vi "Timer_New.vi"(8 "Pass_Through_Time":dbl=-1.0 format="%33.4f") -> (3 "TIMER":T1 {"Accumulated TIme" format="%13.5p"; "StartTime" format="%13.5p"})   [LabVIEW 2019, in "Trajectory_Library.lvlib"]
doc: "Creates and initializes a Timer data cluster.\n\nOutputs:\n - Timer -- The initialized Timer data cluster"
uses:
  Trajectory_Library.lvlib
  TypeDef/TIMER.ctl
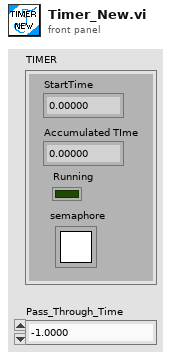
[diagram p1: front panel]
types:
  T1 = typedef "Trajectory_Library.lvlib/TIMER.ctl" = cluster{"StartTime":dbl, "Accumulated TIme":dbl, "Running":bool, "semaphore":T2}
  T2 = typedef "Semaphore RefNum" = refnum<k1>
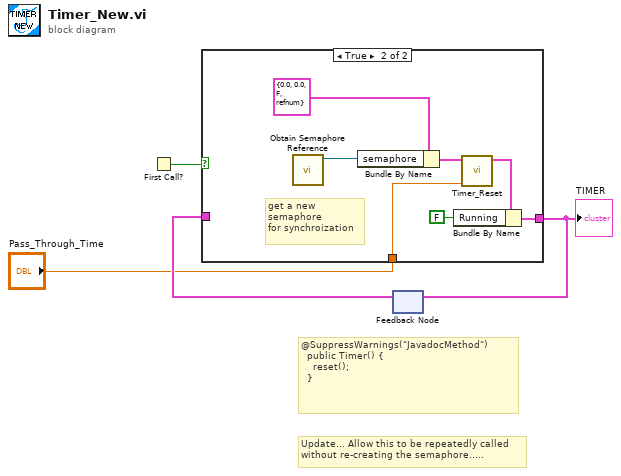
[diagram p0: block diagram]
diagram:
  # "Update... Allow this to be repeatedly called\nwithout re-creating the semaphore....."
  # "@SuppressWarnings(\"JavadocMethod\")\n  public Timer() {\n    reset();\n  }"
  n1 = First Call?() -> (First Call?: T/F=w3:bool)
  n2 = feedback #1() -> (w2:T1)  [unwired: 1 in]
  n3 = case shown="True" w3 {
    tunnel: [w5 w7] -> w4
    tunnel: w2 -> [w5 _]
    tunnel: "Pass_Through_Time" -> [_ w6]
    frame False {
    }
    frame True {
      # "get a new \nsemaphore\nfor synchroization"
      n4 = call <vilib>:"Obtain Semaphore Reference.vi"() -> ("semaphore"=w8:T2)  [unwired: 5 in, 2 out]
      n5 = Bundle By Name(cluster=T1 {"StartTime"=0.0, "Accumulated TIme"=0.0, "Running"=FALSE, "semaphore"=refnum} ("in TIMER"), "semaphore"=w8) -> (w9:T1)
      n6 = call "Timer_Reset.vi"("Pass_Through_Time"=w6, "in TIMER"=w9) -> ("out TIMER"=w12:T1)  [unwired: 9 in]
      n7 = Bundle By Name(cluster=w12, "Running"=FALSE) -> (w7:T1)
    }
  }
  "TIMER" <- w4
  n8 = feedback-in #1(w4) -> ()
